vi "Get Visible State.vi"(8 "error in (no error)":errorcluster, 11 "JKI SM in":refnum<class "JKI SM.lvclass">) -> (0 "error out":errorcluster, 1 "State Name":string, 2 "Category":string, 3 "JKI SM out":refnum<class "JKI SM.lvclass">, 4 "is a Category Frame?":bool, 5 "Idle Frame?":bool)   [LabVIEW 2020, in "JKI State Machine API.lvlib" / "JKI SM.lvclass"]
uses:
  JKI SM.lvclass
  JKI SM.lvclass/JKI SM.ctl
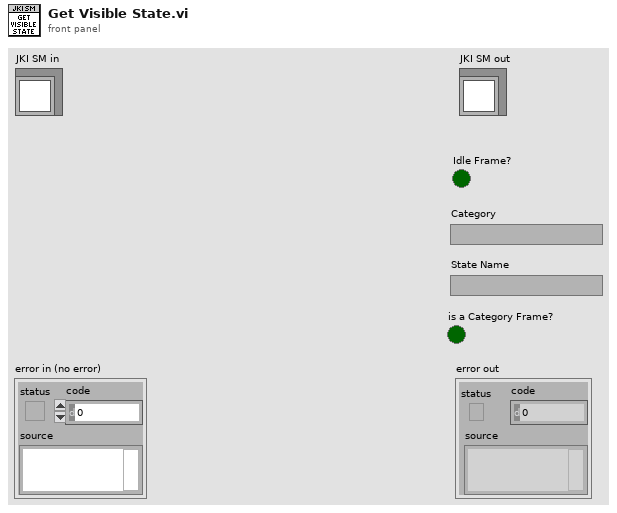
[diagram p1: front panel]
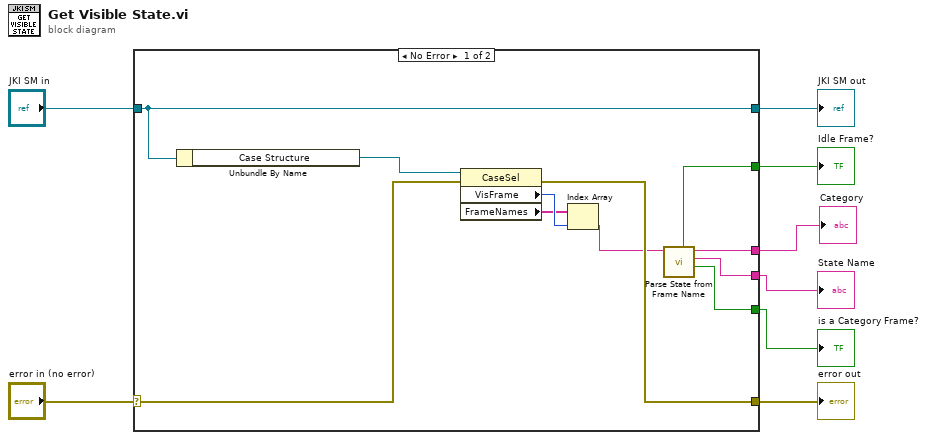
[diagram p0: block diagram]
diagram:
  n1 = case shown="No Error" "error in (no error)" {
    selector: "error in (no error)" -> [w16 w21]
    tunnel: [w19 w21] -> w7
    tunnel: [w17 w20] -> w5
    tunnel: "JKI SM in" -> [w17 w20]
    tunnel: [w12 _] -> w4
    tunnel: [w11 _] -> w3
    tunnel: [w10 _] -> w2
    tunnel: [w9 _] -> w1
    frame No Error {
      n2 = Unbundle By Name(w17) -> ("Case Structure"=w18:refnum<vi>)
      n3 = property class="CaseSel"(reference=w18, error in=w16) -> (error out=w19:errorcluster, "VisFrame"=w15:u32, "FrameNames"=w14:string[])  [unwired: 1 out]
      n4 = Index Array(array=w14, index=w15) -> (element=w13:string)
      n5 = call "Parse State from Frame Name.vi"("Frame or State Name"=w13) -> ("is a Category Frame?"=w10:bool, "State Name"=w11:string, "Category Name"=w12:string, "Idle Frame?"=w9:bool)  [unwired: 5 in, 2 out]
    }
    frame Error {
    }
  }
  "error out" <- w7
  "JKI SM out" <- w5
  "State Name" <- w3
  "Category" <- w4
  "is a Category Frame?" <- w2
  "Idle Frame?" <- w1
